vi "OBCP.vi"() -> ()   [LabVIEW 2019]
uses:
  <vilib>/Instr/_visa.llb/VISA Flush IO Buffer Mask.ctl
  <vilib>/Instr/_visa.llb/VISA Configure Serial Port (Instr).vi
panel:
  out "Acceleration":cluster{"Z":dbl, "Y":dbl, "X":dbl}(graph)
  out "Temperature":i32(graph)
  out "Temperature":i32 format="%d°C"
  in  "Clear":bool
  out "Z":dbl
  out "Y":dbl
  out "X":dbl
  in  "Moteur PWM":u16(slide) step=1 scale=0.0..65535.0
  in  "Led Verte":u16(slide) scale=0.0..65535.0
  in  "Led Rouge":u16(slide) scale=0.0..65535.0
  out "Chaîne":string
  in  "Led Bleu":u16(slide) scale=0.0..65535.0
  in  "Quitter":bool
  in  "Connect":bool
  in  "Port COM":refnum<visa-resource-name> caption="Nom de ressource VISA"
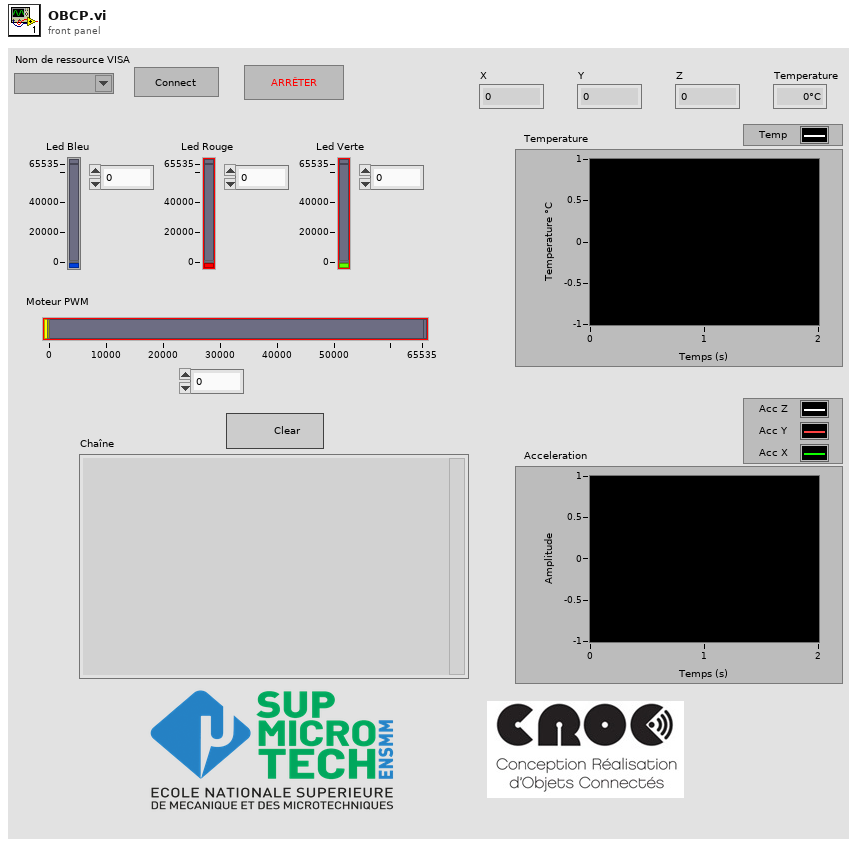
[diagram p1: front panel]
types:
  T1 = typedef "VISA Flush IO Buffer Mask.ctl" = u16
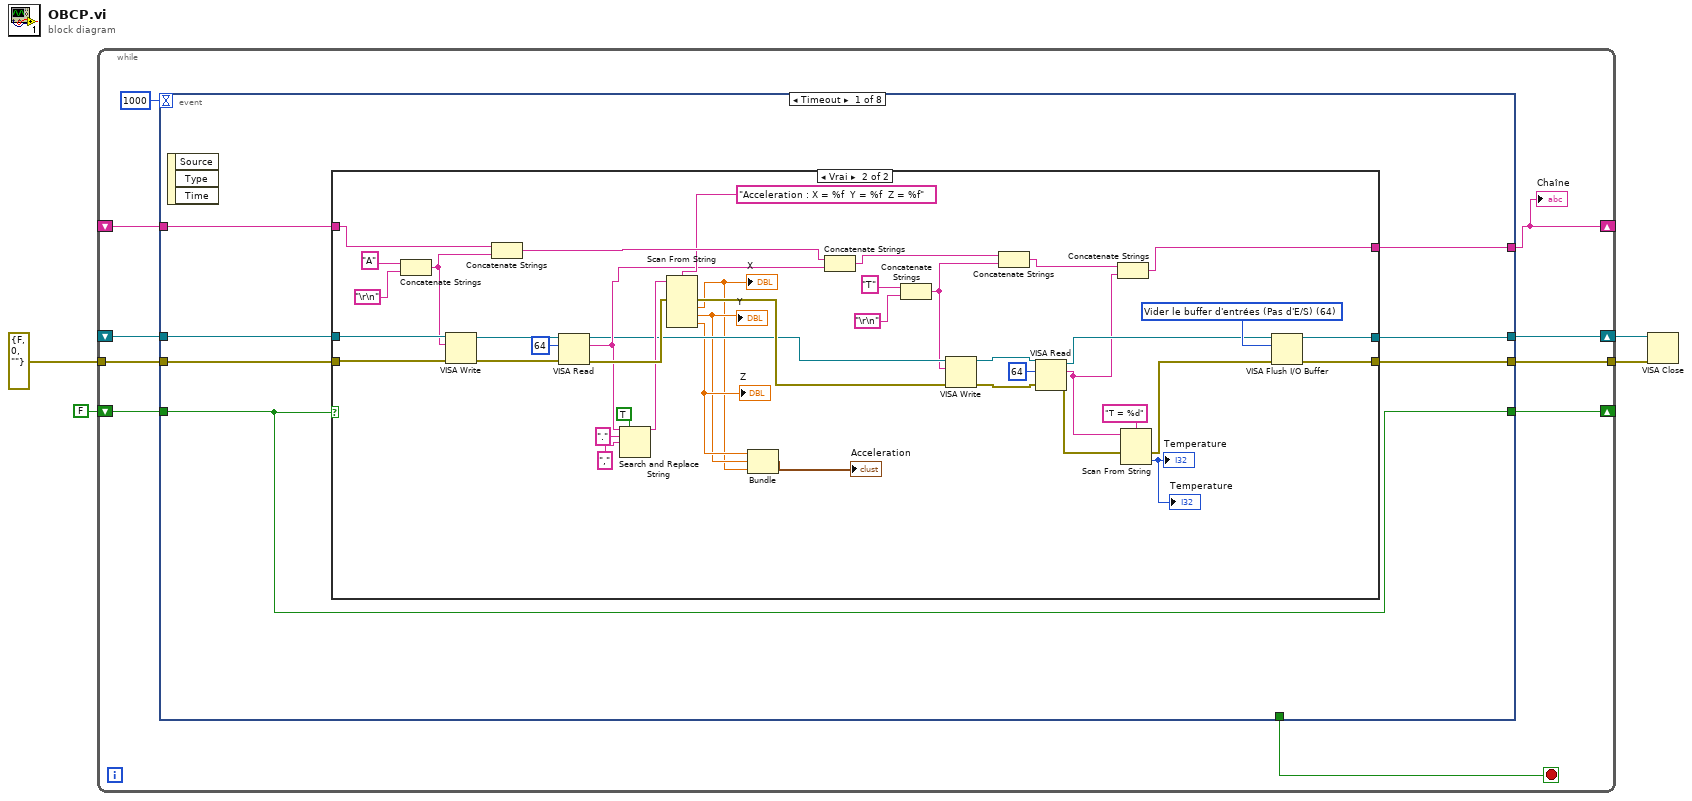
[diagram p0: block diagram]
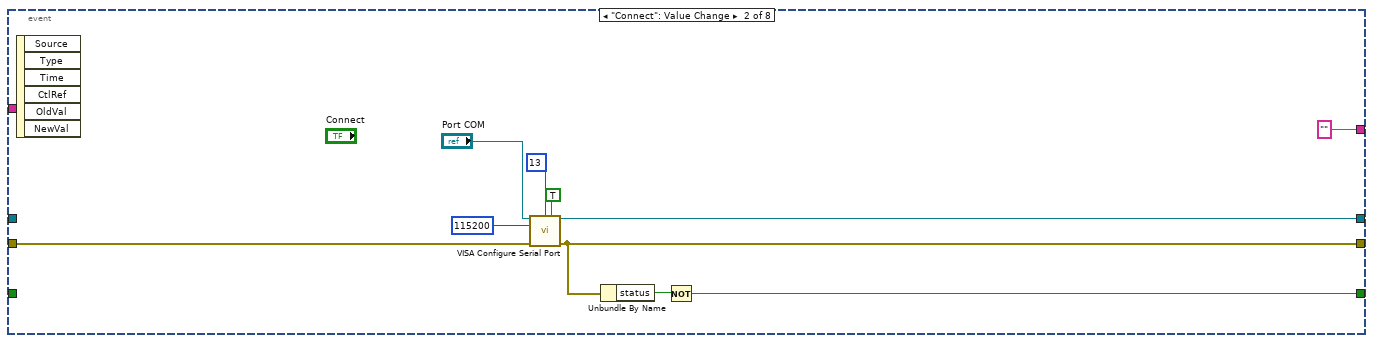
[diagram p3: hidden frame]
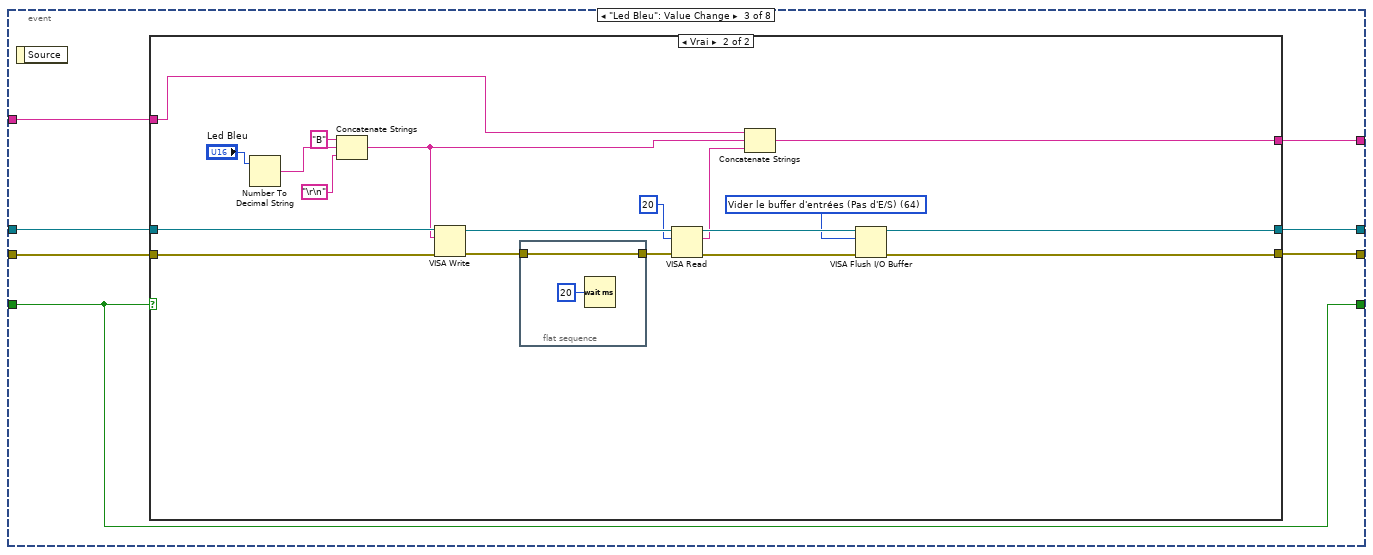
[diagram p4: hidden frame]
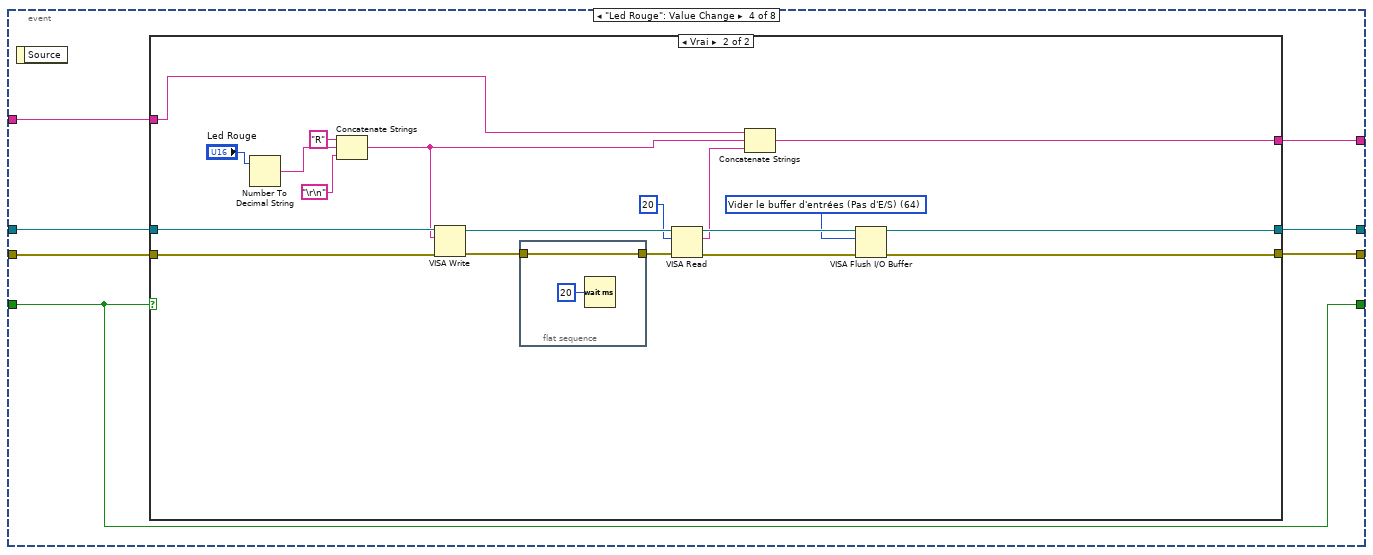
[diagram p6: hidden frame]
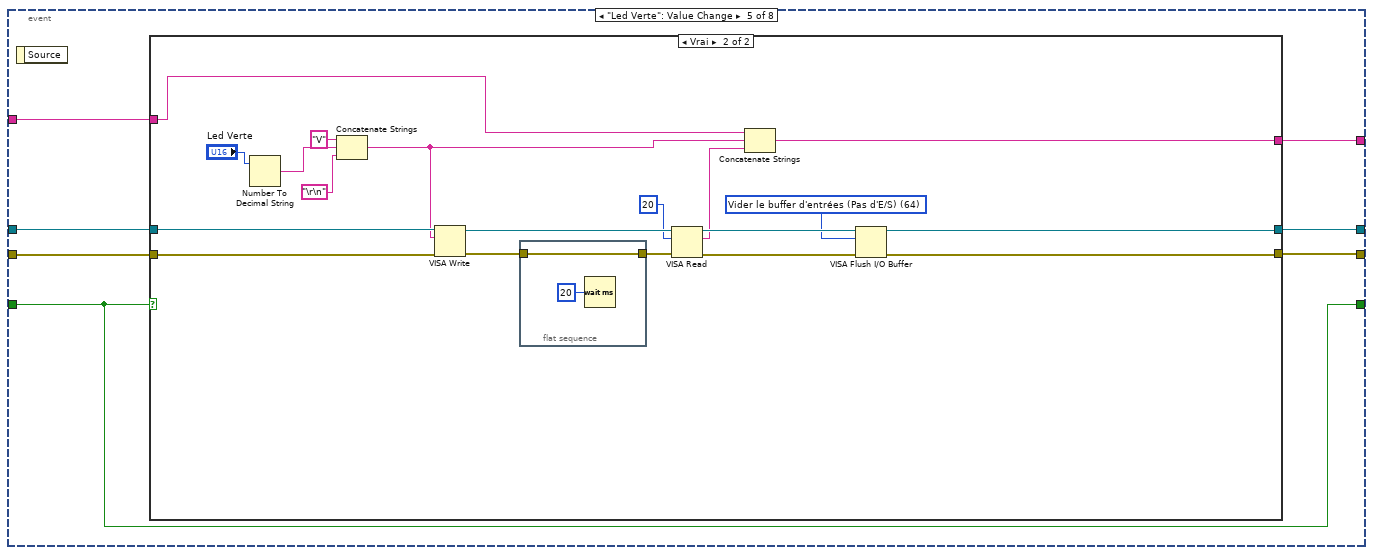
[diagram p8: hidden frame]
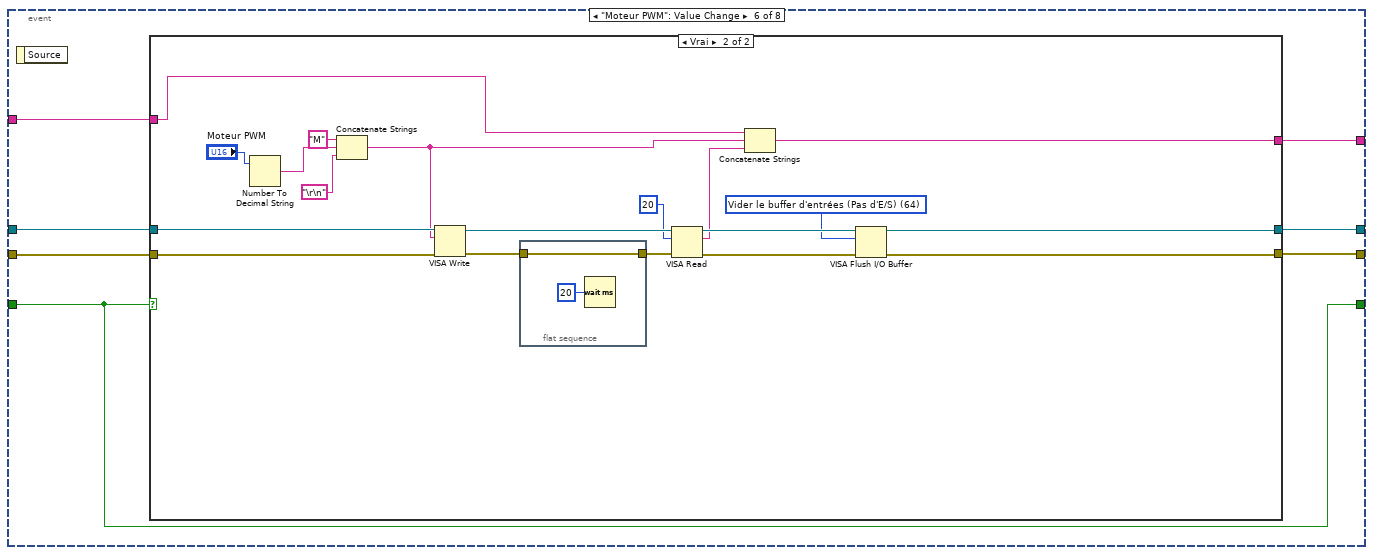
[diagram p10: hidden frame]
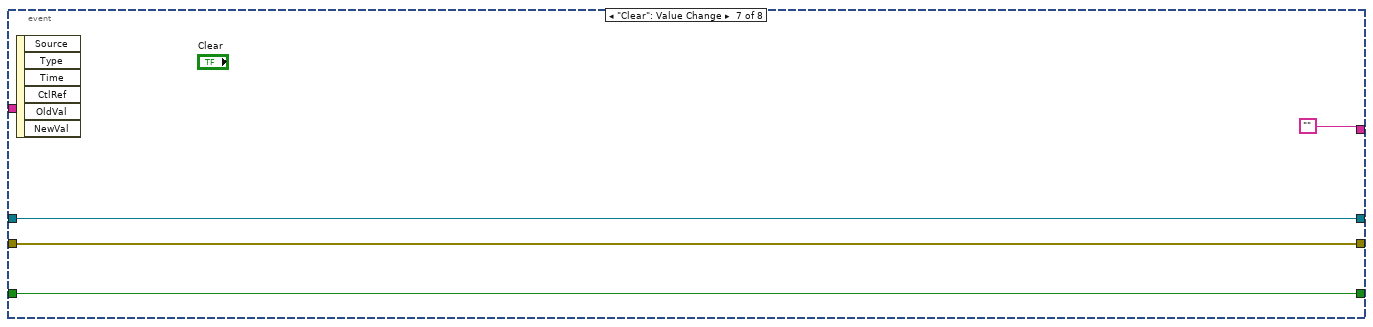
[diagram p12: hidden frame]
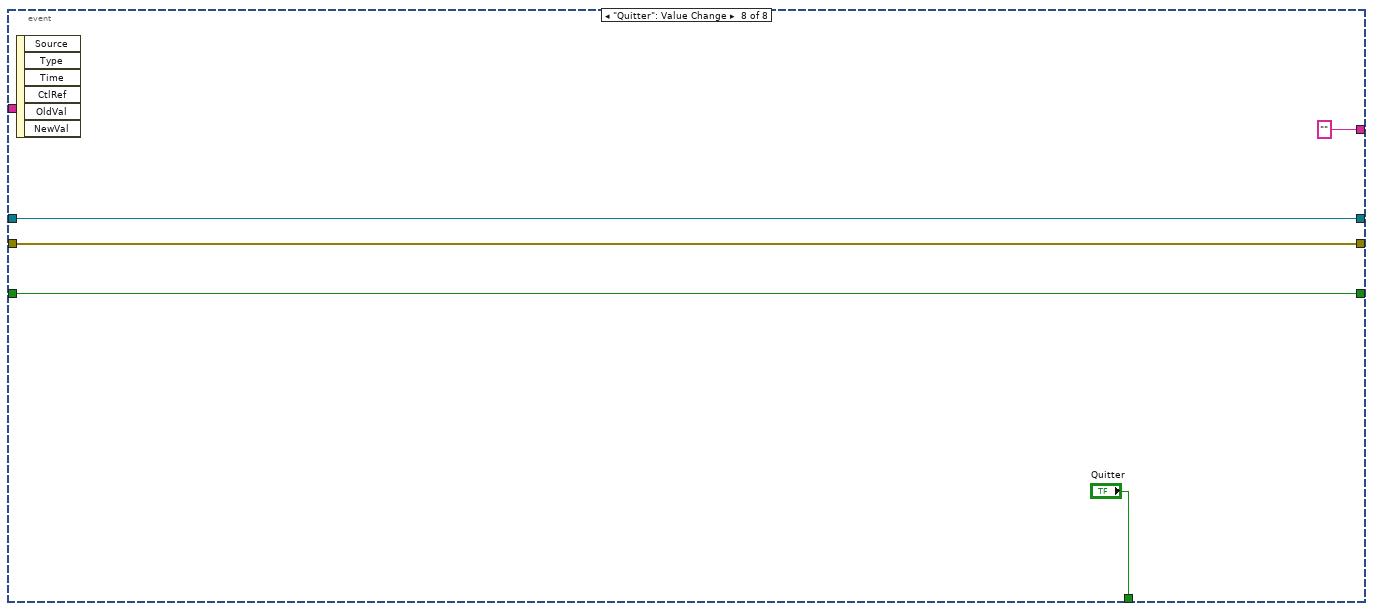
[diagram p13: hidden frame]
diagram:
  n1 = while {
    shift-right: [w14] -> w2
    shift-left: _ -> [w13]
    tunnel: errorcluster {"status"=FALSE, "code"=0, "source"=""} ("constante d'erreur") -> [w12]
    shift-right: [w11] -> _
    shift-left: FALSE -> [w10]
    tunnel: [w8] -> w1
    shift-right: [w6] -> _
    shift-left: _ -> [w5]
    stop <- w7 stop-if-true
    n2 = event shown="[0] Timeout" {
      selector: _ -> [_ _ _ _ _ _ _ _]
      dyn-events: _ -> [_ _ _ _ _ _ _ _]
      timeout: 1000 -> [_ _ _ _ _ _ _ _]
      tunnel: [w19 w74 w79 w110 w141 w172 w203 w208] -> w14
      tunnel: w13 -> [w21 _ w81 w112 w143 w174 w203 w208]
      tunnel: w12 -> [w20 w73 w82 w113 w144 w175 w202 w207]
      tunnel: [w17 w70 w78 w109 w140 w171 w201 w206] -> w11
      tunnel: w10 -> [w17 _ w78 w109 w140 w171 w201 w206]
      tunnel: [w18 w69 w80 w111 w142 w173 w202 w207] -> w8
      tunnel: [_ _ _ _ _ _ _ "Quitter"] -> w7
      tunnel: [w15 "" w77 w108 w139 w170 "" ""] -> w6
      tunnel: w5 -> [w16 _ w76 w107 w138 w169 _ _]
      event Timeout {
        n3 = event-data() -> ()  [unwired: 1 in, 3 out]
        n4 = case shown="Vrai" w17 {
          tunnel: w21 -> [w24 w65]
          tunnel: w20 -> [w23 w64]
          tunnel: [w24 w62] -> w19
          tunnel: [w23 w61] -> w18
          tunnel: w16 -> [w22 w57]
          tunnel: [w22 w29] -> w15
          frame False {
          }
          frame True {
            w63 = T1 64 items=["Vider le buffer d'entrées"=16, "Écrire le buffer de sorties sur le périphérique"=32, "Vider le buffer d'entrées (Pas d'E/S)"=64, "Vider le buffer de sorties"=128] ("Mask")
            n5 = Concatenate Strings("A" ("buffer d'écriture"), "\r\n") -> (w56:string)
            n6 = VISA Write(VISA resource name=w65, write buffer=w56, error in (no error)=w64) -> (VISA resource name out=w55:refnum<visa-resource-name>, error out=w58:errorcluster)  [unwired: 1 out]
            n7 = Concatenate Strings(w57, w56) -> (w53:string)
            n8 = VISA Read(VISA resource name=w55, byte count=u32 64 ("nombre d'octets"), error in (no error)=w58) -> (VISA resource name out=w42:refnum<visa-resource-name>, read buffer=w46:string, error out=w52:errorcluster)  [unwired: 1 out]
            n9 = Search and Replace String(replace all?=TRUE ("tout remplacer ? (F)"), input string=w46, search string="." ("chaîne recherchée"), replace string="," ("chaîne recherchée")) -> (result string=w47:string)  [unwired: 4 in, 3 out]
            n10 = Scan From String(format string="Acceleration : X = %f  Y = %f  Z = %f" ("chaîne de format"), input string=w47, error in=w52) -> (error out=w43:errorcluster, output 1=w26:dbl, output 2=w27:dbl, output 3=w28:dbl)  [unwired: 4 in, 2 out]
            "X" <- w26
            "Y" <- w27
            "Z" <- w28
            n11 = Bundle("Z"=w28, "Y"=w27, "X"=w26) -> (→"Acceleration":cluster{"Z":dbl, "Y":dbl, "X":dbl})  [unwired: 1 in]
            n12 = Concatenate Strings(w53, w46) -> (w33:string)
            n13 = Concatenate Strings("T" ("buffer d'écriture"), "\r\n") -> (w32:string)
            n14 = VISA Write(VISA resource name=w42, write buffer=w32, error in (no error)=w43) -> (VISA resource name out=w40:refnum<visa-resource-name>, error out=w39:errorcluster)  [unwired: 1 out]
            n15 = Concatenate Strings(w33, w32) -> (w31:string)
            n16 = VISA Read(VISA resource name=w40, byte count=u32 64 ("nombre d'octets"), error in (no error)=w39) -> (VISA resource name out=w38:refnum<visa-resource-name>, read buffer=w30:string, error out=w36:errorcluster)  [unwired: 1 out]
            n17 = Concatenate Strings(w31, w30) -> (w29:string)
            n18 = Scan From String(format string="T = %d" ("chaîne de format"), input string=w30, error in=w36) -> (error out=w35:errorcluster, output 1=→"Temperature" →"Temperature":i32)  [unwired: 2 in, 2 out]
            n19 = VISA Flush I/O Buffer(VISA resource name=w38, mask (16)=w63, error in (no error)=w35) -> (VISA resource name out=w62:refnum<visa-resource-name>, error out=w61:errorcluster)
          }
        }
      }
      event "Connect": Value Change {
        n20 = event-data() -> ()  [unwired: 1 in, 6 out]
        n21 = call-poly "VISA Configure Serial Port"("VISA resource name"="Port COM", "termination char\n(0xA = '\\n' = LF)"=u8 13 ("termination char\n(0xA = '\\n' = LF)"), "Enable Termination\nChar (T)"=TRUE ("Enable Termination\nChar (T)"), "baud rate (9600)"=u32 115200, "error in (no error)"=w73) -> ("VISA resource name out"=w74:refnum<visa-resource-name>, "error out"=w69:errorcluster)  [unwired: 9 in]
        n22 = Unbundle By Name(w69) -> ("status"=w71:bool)
        n23 = Not(x=w71) -> (.not. x?=w70:bool)
      }
      event "Led Bleu": Value Change {
        n24 = event-data() -> ()  [unwired: 1 in, 1 out]
        n25 = case shown="Vrai" w78 {
          tunnel: w82 -> [w84 w104]
          tunnel: w81 -> [w85 w100]
          tunnel: [w84 w95] -> w80
          tunnel: [w85 w96] -> w79
          tunnel: [w83 w87] -> w77
          tunnel: w76 -> [w83 w86]
          frame False {
          }
          frame True {
            w97 = T1 64 items=["Vider le buffer d'entrées"=16, "Écrire le buffer de sorties sur le périphérique"=32, "Vider le buffer d'entrées (Pas d'E/S)"=64, "Vider le buffer de sorties"=128] ("Mask")
            n26 = Number To Decimal String(number="Led Bleu") -> (decimal integer string=w90:string)  [unwired: 1 in]
            n27 = Concatenate Strings("B" ("chaîne"), w90, "\r\n") -> (w88:string)
            n28 = VISA Write(VISA resource name=w100, write buffer=w88, error in (no error)=w104) -> (VISA resource name out=w101:refnum<visa-resource-name>, error out=w103:errorcluster)  [unwired: 1 out]
            n29 = flat-sequence {
              tunnel: w103 -> [w106]
              tunnel: [w106] -> w102
              frame #0 {
                n30 = Wait (ms)(milliseconds to wait=u32 20 ("attente (ms)")) -> ()  [unwired: 1 out]
              }
            }
            n31 = VISA Read(VISA resource name=w101, byte count=u32 20 ("nombre d'octets"), error in (no error)=w102) -> (VISA resource name out=w99:refnum<visa-resource-name>, read buffer=w93:string, error out=w98:errorcluster)  [unwired: 1 out]
            n32 = Concatenate Strings(w86, w88, w93) -> (w87:string)
            n33 = VISA Flush I/O Buffer(VISA resource name=w99, mask (16)=w97, error in (no error)=w98) -> (VISA resource name out=w96:refnum<visa-resource-name>, error out=w95:errorcluster)
          }
        }
      }
      event "Led Rouge": Value Change {
        n34 = event-data() -> ()  [unwired: 1 in, 1 out]
        n35 = case shown="Vrai" w109 {
          tunnel: w113 -> [w115 w135]
          tunnel: w112 -> [w116 w131]
          tunnel: [w115 w126] -> w111
          tunnel: [w116 w127] -> w110
          tunnel: [w114 w118] -> w108
          tunnel: w107 -> [w114 w117]
          frame False {
          }
          frame True {
            w128 = T1 64 items=["Vider le buffer d'entrées"=16, "Écrire le buffer de sorties sur le périphérique"=32, "Vider le buffer d'entrées (Pas d'E/S)"=64, "Vider le buffer de sorties"=128] ("Mask")
            n36 = Number To Decimal String(number="Led Rouge") -> (decimal integer string=w121:string)  [unwired: 1 in]
            n37 = Concatenate Strings("R" ("chaîne"), w121, "\r\n") -> (w119:string)
            n38 = VISA Write(VISA resource name=w131, write buffer=w119, error in (no error)=w135) -> (VISA resource name out=w132:refnum<visa-resource-name>, error out=w134:errorcluster)  [unwired: 1 out]
            n39 = flat-sequence {
              tunnel: w134 -> [w137]
              tunnel: [w137] -> w133
              frame #0 {
                n40 = Wait (ms)(milliseconds to wait=u32 20 ("attente (ms)")) -> ()  [unwired: 1 out]
              }
            }
            n41 = VISA Read(VISA resource name=w132, byte count=u32 20 ("nombre d'octets"), error in (no error)=w133) -> (VISA resource name out=w130:refnum<visa-resource-name>, read buffer=w124:string, error out=w129:errorcluster)  [unwired: 1 out]
            n42 = Concatenate Strings(w117, w119, w124) -> (w118:string)
            n43 = VISA Flush I/O Buffer(VISA resource name=w130, mask (16)=w128, error in (no error)=w129) -> (VISA resource name out=w127:refnum<visa-resource-name>, error out=w126:errorcluster)
          }
        }
      }
      event "Led Verte": Value Change {
        n44 = event-data() -> ()  [unwired: 1 in, 1 out]
        n45 = case shown="Vrai" w140 {
          tunnel: w144 -> [w146 w166]
          tunnel: w143 -> [w147 w162]
          tunnel: [w146 w157] -> w142
          tunnel: [w147 w158] -> w141
          tunnel: [w145 w149] -> w139
          tunnel: w138 -> [w145 w148]
          frame False {
          }
          frame True {
            w159 = T1 64 items=["Vider le buffer d'entrées"=16, "Écrire le buffer de sorties sur le périphérique"=32, "Vider le buffer d'entrées (Pas d'E/S)"=64, "Vider le buffer de sorties"=128] ("Mask")
            n46 = Number To Decimal String(number="Led Verte") -> (decimal integer string=w152:string)  [unwired: 1 in]
            n47 = Concatenate Strings("V" ("chaîne"), w152, "\r\n") -> (w150:string)
            n48 = VISA Write(VISA resource name=w162, write buffer=w150, error in (no error)=w166) -> (VISA resource name out=w163:refnum<visa-resource-name>, error out=w165:errorcluster)  [unwired: 1 out]
            n49 = flat-sequence {
              tunnel: w165 -> [w168]
              tunnel: [w168] -> w164
              frame #0 {
                n50 = Wait (ms)(milliseconds to wait=u32 20 ("attente (ms)")) -> ()  [unwired: 1 out]
              }
            }
            n51 = VISA Read(VISA resource name=w163, byte count=u32 20 ("nombre d'octets"), error in (no error)=w164) -> (VISA resource name out=w161:refnum<visa-resource-name>, read buffer=w155:string, error out=w160:errorcluster)  [unwired: 1 out]
            n52 = Concatenate Strings(w148, w150, w155) -> (w149:string)
            n53 = VISA Flush I/O Buffer(VISA resource name=w161, mask (16)=w159, error in (no error)=w160) -> (VISA resource name out=w158:refnum<visa-resource-name>, error out=w157:errorcluster)
          }
        }
      }
      event "Moteur PWM": Value Change {
        n54 = event-data() -> ()  [unwired: 1 in, 1 out]
        n55 = case shown="Vrai" w171 {
          tunnel: w175 -> [w177 w197]
          tunnel: w174 -> [w178 w193]
          tunnel: [w177 w188] -> w173
          tunnel: [w178 w189] -> w172
          tunnel: [w176 w180] -> w170
          tunnel: w169 -> [w176 w179]
          frame False {
          }
          frame True {
            w190 = T1 64 items=["Vider le buffer d'entrées"=16, "Écrire le buffer de sorties sur le périphérique"=32, "Vider le buffer d'entrées (Pas d'E/S)"=64, "Vider le buffer de sorties"=128] ("Mask")
            n56 = Number To Decimal String(number="Moteur PWM") -> (decimal integer string=w183:string)  [unwired: 1 in]
            n57 = Concatenate Strings("M" ("chaîne"), w183, "\r\n") -> (w181:string)
            n58 = VISA Write(VISA resource name=w193, write buffer=w181, error in (no error)=w197) -> (VISA resource name out=w194:refnum<visa-resource-name>, error out=w196:errorcluster)  [unwired: 1 out]
            n59 = flat-sequence {
              tunnel: w196 -> [w199]
              tunnel: [w199] -> w195
              frame #0 {
                n60 = Wait (ms)(milliseconds to wait=u32 20 ("attente (ms)")) -> ()  [unwired: 1 out]
              }
            }
            n61 = VISA Read(VISA resource name=w194, byte count=u32 20 ("nombre d'octets"), error in (no error)=w195) -> (VISA resource name out=w192:refnum<visa-resource-name>, read buffer=w186:string, error out=w191:errorcluster)  [unwired: 1 out]
            n62 = Concatenate Strings(w179, w181, w186) -> (w180:string)
            n63 = VISA Flush I/O Buffer(VISA resource name=w192, mask (16)=w190, error in (no error)=w191) -> (VISA resource name out=w189:refnum<visa-resource-name>, error out=w188:errorcluster)
          }
        }
      }
      event "Clear": Value Change {
        n64 = event-data() -> ()  [unwired: 1 in, 6 out]
      }
      event "Quitter": Value Change {
        n65 = event-data() -> ()  [unwired: 1 in, 6 out]
      }
    }
    "Chaîne" <- w6
  }
  n66 = VISA Close(VISA resource name=w2, error in (no error)=w1) -> ()  [unwired: 1 out]
